vi "Add Suffix to File Name.vi"(10 "Suffix":string, 11 "File Path in":path) -> (3 "File Path out":path)   [LabVIEW 2026]
doc: "This VI adds the provided suffix to the file name before the file extension."
uses:
  <userlib>/_OpenG.lib/file/file.llb/openg_file.lvlib
  <userlib>/_OpenG.lib/file/file.llb/Convert File Extension (String)__ogtk.vi
  <userlib>/_OpenG.lib/file/file.llb/Strip Path Extension - String__ogtk.vi
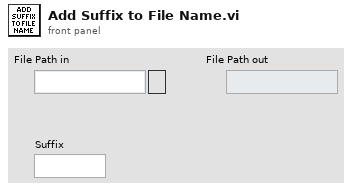
[diagram p1: front panel]
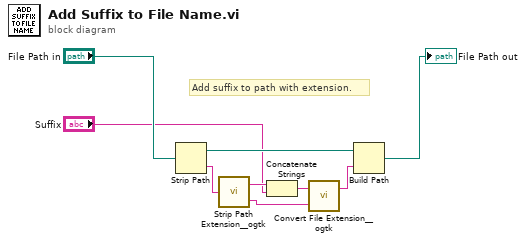
[diagram p0: block diagram]
diagram:
  # "Add suffix to path with extension."
  n1 = Strip Path(path="File Path in") -> (stripped path=w4:path, name=w9:string)
  n2 = call-poly <userlib>:"Strip Path Extension__ogtk.vi"("path"=w9) -> ("root"=w8:string, "extension"=w6:string)
  n3 = Concatenate Strings(w8, "Suffix") -> (w7:string)
  n4 = call-poly <userlib>:"Convert File Extension__ogtk.vi"("new ending (none)"=w6, "file name"=w7) -> ("new filename"=w5:string)  [unwired: 1 out]
  n5 = Build Path(base path=w4, name or relative path=w5) -> (appended path=→"File Path out":path)
